vi "generate table.vi"(4 "Filter":string, 5 "to cvt":refnum<vi>, 6 "Direction":enum32{"From CVT", "To CVT"}(radio), 7 "from cvt":refnum<vi>, 8 "error in":errorcluster, 9 "avail tags":refnum<vi>, 10 "engine configuration in":refnum<class "engine configuration.lvclass">, 11 "cvt in":refnum<class "CVT configuration.lvclass">) -> (0 "error out":errorcluster, 2 "engine configuration out":refnum<class "engine configuration.lvclass">, 3 "cvt out":refnum<class "CVT configuration.lvclass">)   [LabVIEW 2013, in "CVT editor node.lvclass"]
uses:
  CVT editor node.lvclass
  configuration/CVT configuration.lvclass
  <vilib>/NI/Module Execution Interface/Engine Configuration/engine configuration.lvclass
  <vilib>/NI/Configuration Framework/serializable configuration/NISE_CEF_serializable configuration.lvclass/NISE_CEF_serializable configuration.ctl
  configuration/CVT configuration.lvclass/CVT configuration.ctl
  <vilib>/NI/Tag Bus/tag/tag descriptor.lvclass/tag descriptor.ctl
  <vilib>/NI/Tag Bus Module Framework/channel/channel classification.ctl
  <vilib>/NI/Tag Bus Module Framework/channel/TBM channel.lvclass/TBM channel.ctl
  <vilib>/NI/Module Execution Interface/Engine Configuration/engine configuration.lvclass/engine configuration.ctl
  <vilib>/NI/Tag Bus/tag/write tag name.vi
  <vilib>/NI/Tag Bus/tag/read tag name.vi
  <vilib>/NI/Tag Bus Module Framework/channel/Read channel classification.vi
  <vilib>/NI/Tag Bus/tag/read data type.vi
  <vilib>/NI/Configuration Framework/serializable configuration/Read UID.vi
  configuration/Read channels.vi
  Item Names.vi
  Apply Filter_1D.vi
  Apply Filter_2D.vi
  <vilib>/Utility/LVClass/Get LV Class Name.vi
  <vilib>/NI/Configuration Framework/error generator/NISE_error generator.vi
  <vilib>/NI/Tag Bus Module Framework/channel/TBM channel.lvclass
  <vilib>/NI/Tag Bus/tag/tag descriptor.lvclass
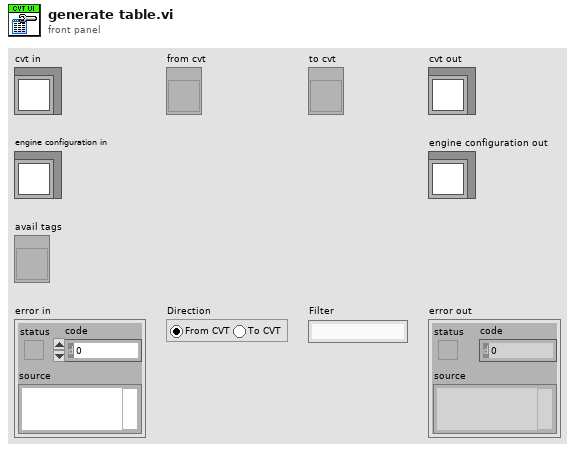
[diagram p1: front panel]
types:
  T1 = typedef "tag bus.lvlib/tag descriptor.lvclass/Data Type.ctl" = enum16{"Double", "Single", "I64", "I32", "I16", "I8", "U64", "U32", "U16", "U8", "Boolean", "String", "Array of Double", "Array of Single", "Array of I64", "Array of I32", "Array of I16", "Array of I8", "Array of U64", "Array of U32", "Array of U16", "Array of U8", "Array of Boolean", "Array of String"}
  T2 = typedef "TBM channel.lvclass/channel classification.ctl" = enum16{"input data", "output data", "processing parameter", "processing result"}
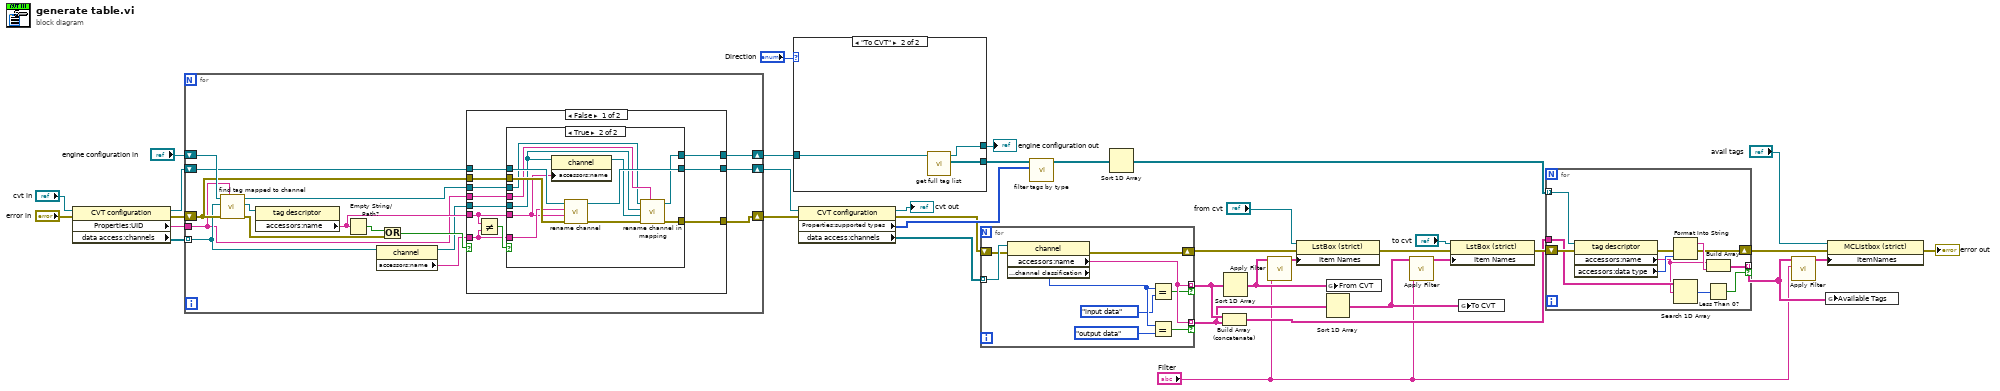
[diagram p0: block diagram]
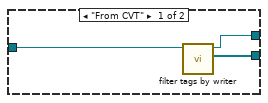
[diagram p2: hidden frame]
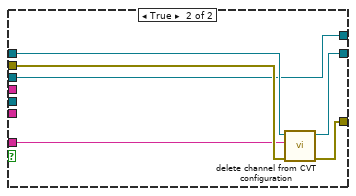
[diagram p4: hidden frame]
diagram:
  n1 = property class="CVT configuration"(reference="cvt in", error in="error in") -> (reference out=w35:refnum<class "CVT configuration.lvclass">, error out=w36:errorcluster, "Properties:UID"=w31:string, "data access:channels"=w37:refnum<class "TBM channel.lvclass">[])
  n2 = for {
    tunnel: w37 -> [w43] mode=indexing
    shift-right: [w38] -> w23
    shift-left: "engine configuration in" -> [w53]
    shift-right: [w50] -> w34
    shift-left: w35 -> [w48]
    tunnel: w31 -> [w40]
    shift-right: [w49] -> w33
    shift-left: w36 -> [w46]
    n3 = call <vilib>:"find tag mapped to channel.vi"("owner"=w40, "error in"=w46, "channel"=w43, "engine configuration in"=w53) -> ("error out"=w45:errorcluster, "tag"=w52:refnum<class "tag descriptor.lvclass">, "engine configuration out"=w39:refnum<class "engine configuration.lvclass">)  [unwired: 5 in]
    n4 = property class="tag descriptor"(reference=w52) -> ("accessors:name"=w42:string)  [unwired: 1 in, 2 out]
    n5 = Empty String/Path?(string/path=w42) -> (empty?=w51:bool)
    n6 = property class="channel"(reference=w43) -> (reference out=w41:refnum<class "TBM channel.lvclass">, "accessors:name"=w44:string)  [unwired: 1 in, 1 out]
    n7 = Or(x=w51, y=w45) -> (x .or. y?=w47:bool)
    n8 = case shown="False" w47 {
      tunnel: [w61 w85] -> w50
      tunnel: [w64 w84] -> w49
      tunnel: w46 -> [w63 w83]
      tunnel: w48 -> [w62 w82]
      tunnel: w44 -> [w59 w81]
      tunnel: w42 -> [w58 _]
      tunnel: w41 -> [w57 _]
      tunnel: w40 -> [w56 _]
      tunnel: w39 -> [w55 w80]
      tunnel: [w54 w80] -> w38
      frame False {
        n9 = Not Equal?(x=w58, y=w59) -> (x != y?=w60:bool)
        n10 = case shown="True" w60 {
          tunnel: [w67 w74] -> w64
          tunnel: w63 -> [w67 w79]
          tunnel: w62 -> [w66 w78]
          tunnel: [w66 w77] -> w61
          tunnel: w59 -> [_ w76]
          tunnel: w58 -> [_ w73]
          tunnel: w57 -> [_ w72]
          tunnel: w56 -> [_ w70]
          tunnel: w55 -> [w65 w69]
          tunnel: [w65 w68] -> w54
          frame False {
          }
          frame True {
            n11 = property class="channel"(reference=w72, "accessors:name"=w73) -> (reference out=w71:refnum<class "TBM channel.lvclass">)  [unwired: 1 in, 1 out]
            n12 = call "rename channel.vi"("error in"=w79, "new name"=w73, "old name"=w76, "CVT configuration in"=w78) -> ("error out"=w75:errorcluster, "CVT configuration out"=w77:refnum<class "CVT configuration.lvclass">)  [unwired: 6 in]
            n13 = call <vilib>:"rename channel in mapping.vi"("owner ID"=w70, "error in"=w75, "new channel"=w71, "old channel"=w72, "engine configuration in"=w69) -> ("error out"=w74:errorcluster, "engine configuration out"=w68:refnum<class "engine configuration.lvclass">)  [unwired: 5 in]
          }
        }
      }
      frame True {
        n14 = call "delete channel from CVT configuration.vi"("error in"=w83, "channel to delete"=w81, "CVT configuration in"=w82) -> ("error out"=w84:errorcluster, "CVT configuration out"=w85:refnum<class "CVT configuration.lvclass">)  [unwired: 7 in]
      }
    }
  }
  n15 = case shown="\"To CVT\"" "Direction" {
    tunnel: w23 -> [w88 w91]
    tunnel: [w87 w90] -> w22
    tunnel: [w86 w89] -> w8
    frame "From CVT" {
      n16 = call <vilib>:"filter tags by writer.vi"("engine configuration in"=w88) -> ("tag list"=w87:refnum<class "tag descriptor.lvclass">[], "engine configuration out"=w86:refnum<class "engine configuration.lvclass">)  [unwired: 9 in]
    }
    frame "To CVT" {
      n17 = call <vilib>:"get full tag list.vi"("engine configuration in"=w91) -> ("tag list"=w90:refnum<class "tag descriptor.lvclass">[], "engine configuration out"=w89:refnum<class "engine configuration.lvclass">)  [unwired: 9 in]
    }
  }
  "engine configuration out" <- w8
  n18 = property class="CVT configuration"(reference=w34, error in=w33) -> (reference out=→"cvt out":refnum<class "CVT configuration.lvclass">, error out=w29:errorcluster, "Properties:supported types"=w32:T1[], "data access:channels"=w30:refnum<class "TBM channel.lvclass">[])
  n19 = for {
    tunnel: w30 -> [w100] mode=indexing
    shift-right: [w99] -> w16
    shift-left: w29 -> [w98]
    tunnel: [w97] -> w12 mode=indexing if=w95
    tunnel: [w97] -> w13 mode=indexing if=w94
    n20 = property class="channel"(reference=w100, error in=w98) -> (error out=w99:errorcluster, "accessors:name"=w97:string, "data access:channel classification"=w96:T2)  [unwired: 1 out]
    n21 = Equal?(x=w96, y=channel_classification."input data") -> (x = y?=w94:bool)
    n22 = Equal?(x=w96, y=channel_classification."output data") -> (x = y?=w95:bool)
  }
  n23 = call <vilib>:"filter tags by type.vi"("allowable types"=w32, "tags in"=w22) -> ("filtered tags"=w28:refnum<class "tag descriptor.lvclass">[])  [unwired: 9 in]
  n24 = Sort 1D Array(array=w28) -> (sorted array=w9:refnum<class "tag descriptor.lvclass">[])
  n25 = Build Array (concatenate)(w13, w12) -> (w11:string[])
  n26 = Sort 1D Array(array=w13) -> (sorted array=w5:string[])
  n27 = call-poly "Apply Filter.vi"("Filter"="Filter", "Item names"=w5) -> ("Filtered Item Names"=w4:string[])  [unwired: 9 in]
  n28 = property class="LstBox (strict)"(reference="from cvt", error in=w16, "Item Names"=w4) -> (error out=w15:errorcluster)  [unwired: 1 out]
  n29 = global write "Item Names.vi" "From CVT"(w5) -> ()
  n30 = Sort 1D Array(array=w12) -> (sorted array=w6:string[])
  n31 = call-poly "Apply Filter.vi"("Filter"="Filter", "Item names"=w6) -> ("Filtered Item Names"=w7:string[])  [unwired: 9 in]
  n32 = property class="LstBox (strict)"(reference="to cvt", error in=w15, "Item Names"=w7) -> (error out=w27:errorcluster)  [unwired: 1 out]
  n33 = global write "Item Names.vi" "To CVT"(w6) -> ()
  n34 = for {
    tunnel: w9 -> [w109] mode=indexing
    shift-right: [w106] -> w26
    shift-left: w27 -> [w108]
    tunnel: [w105] -> w3 mode=indexing if=w101
    tunnel: w11 -> [w104]
    n35 = property class="tag descriptor"(reference=w109, error in=w108) -> (error out=w107:errorcluster, "accessors:name"=w102:string, "accessors:data type"=w110:T1)  [unwired: 1 out]
    n36 = Format Into String(error in=w107, w110) -> (resulting string=w111:string, error out=w106:errorcluster)  [unwired: 2 in]
    n37 = Search 1D Array(1D array=w104, element=w102) -> (index of element=w103:i32)  [unwired: 1 in]
    n38 = Less Than 0?(x=w103) -> (x < 0?=w101:bool)
    n39 = Build Array(w102, w111) -> (w105:string[])
  }
  n40 = call-poly "Apply Filter.vi"("Filter"="Filter", "Item names"=w3) -> ("Filtered Item Names"=w2:string[][])  [unwired: 9 in]
  n41 = global write "Item Names.vi" "Available Tags"(w3) -> ()
  n42 = property class="MCListbox (strict)"(reference="avail tags", error in=w26, "ItemNames"=w2) -> (error out=→"error out":errorcluster)  [unwired: 1 out]
